vi "Find All Referenced Structures.vi"(8 "error in":errorcluster, 11 "ParseGDSII in":refnum<class "ParseGDSII.lvclass">) -> (0 "error out":errorcluster, 3 "ParseGDSII out":refnum<class "ParseGDSII.lvclass">)   [LabVIEW 2019, in "ParseGDSII.lvclass"]
uses:
  ParseGDSII.lvclass
  Fast Tree/Fast Tree.lvclass
  920f742c-f628-416c-89cb-44049b089101.vi
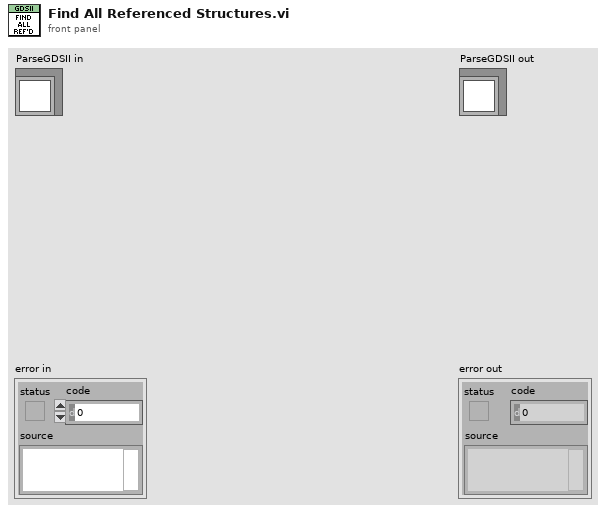
[diagram p1: front panel]
types:
  T1 = cluster{"Record Type":string, "Payload":string, "Parent Index":i32, "First Child Index":i32, "Next Sibling Index":i32}[]
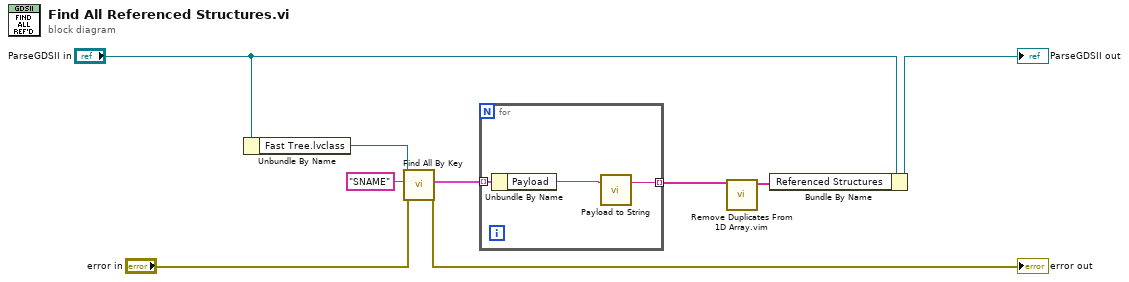
[diagram p0: block diagram]
diagram:
  n1 = Unbundle By Name("ParseGDSII in") -> ("Fast Tree.lvclass"=w5:refnum<class "Fast Tree.lvclass">)
  n2 = call "Find All By Key.vi"("error in"="error in", "Key"="SNAME", "Fast Tree in"=w5) -> ("error out"=→"error out":errorcluster, "Found Items"=w4:T1)  [unwired: 6 in, 1 out]
  n3 = for {
    tunnel: w4 -> [w12] mode=indexing
    tunnel: [w10] -> w3 mode=indexing
    n4 = Unbundle By Name(w12) -> ("Payload"=w11:string)
    n5 = call "Payload to String.vi"("Payload"=w11) -> ("String"=w10:string)  [unwired: 2 in]
  }
  n6 = call "Remove Duplicates From 1D Array.vim"("array"=w3) -> ("array with duplicates removed"=w2:string[])  [unwired: 10 in]
  n7 = Bundle By Name(cluster="ParseGDSII in", "Referenced Structures"=w2) -> (→"ParseGDSII out":refnum<class "ParseGDSII.lvclass">)
